vi "Connect-string.vi"(8 "error in (no error)":errorcluster caption="错误输入（无错误）", 10 "database-path":path, 11 "Database_access 输入":refnum<class "Database_access.lvclass">) -> (0 "error out":errorcluster caption="错误输出", 2 "connection reference":T1, 3 "Database_access 输出":refnum<class "Database_access.lvclass">)   [LabVIEW 2025, in "Database_access.lvclass"]
uses:
  Database_access.lvclass
  <vilib>/addons/database/Connection.llb/Conn ObjectReference.ctl
  Database_access.lvclass/Database_access.ctl
  <vilib>/addons/database/Connection.llb/DB Tools Open Connec (String).vi
  <vilib>/regexp/Match Regular Expression.xnode
  <vilib>/addons/database/NI_Database_API.lvlib
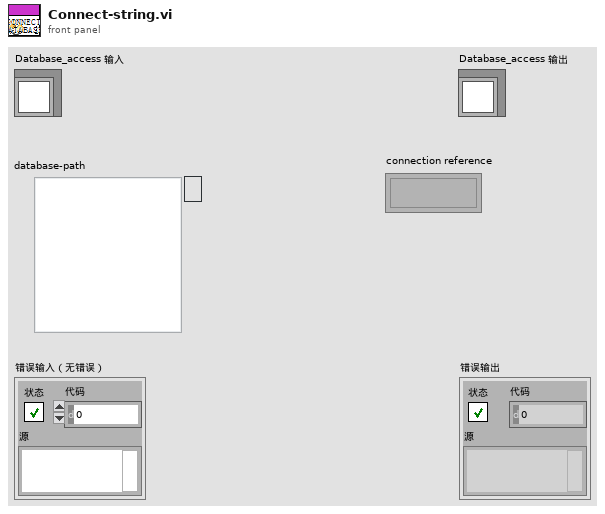
[diagram p1: front panel]
types:
  T1 = typedef "NI_Database_API.lvlib/Conn ObjectReference.ctl" = refnum<k1>
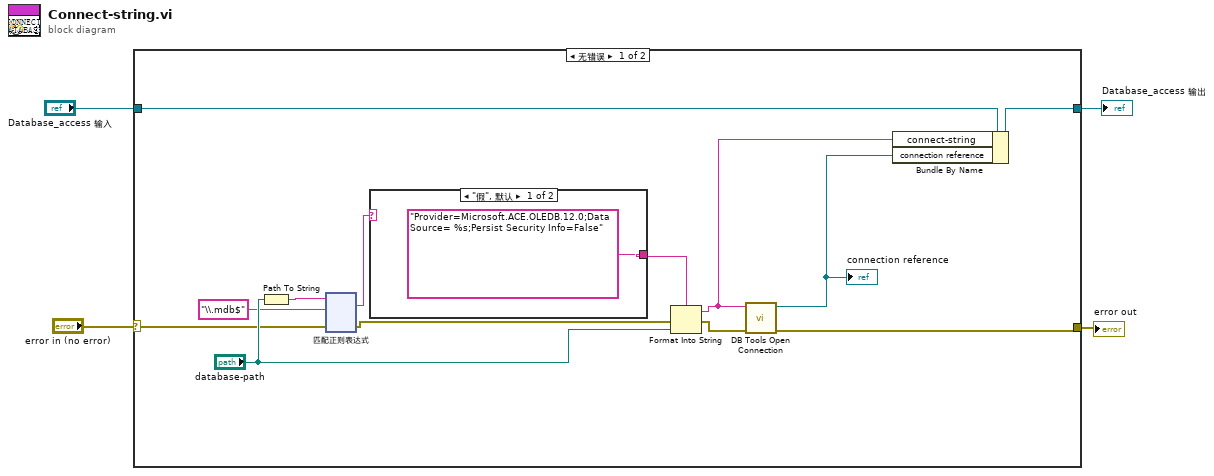
[diagram p0: block diagram]
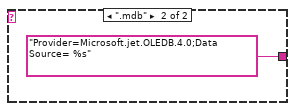
[diagram p2: hidden frame]
diagram:
  n1 = case shown="无错误" "error in (no error)" {
    selector: "error in (no error)" -> [w10 w138]
    tunnel: [w5 w138] -> w3
    tunnel: [w16 w137] -> w1
    tunnel: "Database_access 输入" -> [w17 w137]
    frame No Error {
      n2 = Path To String(path="database-path") -> (string=w12:string)
      n3 = xnode "匹配正则表达式"("输入字符串"=w12, "正则表达式"="\\.mdb$", "错误输入"=w10) -> ("所有匹配"=w9:string, "错误输出"=w8:errorcluster)  [unwired: 3 in, 3 out]
      n4 = case shown="\"假\", 默认" w9 {
        tunnel: ["Provider=Microsoft.ACE.OLEDB.12.0;Data Source= %s;Persist Security Info=False" "Provider=Microsoft.jet.OLEDB.4.0;Data Source= %s"] -> w7
        frame "假", Default {
        }
        frame ".mdb" {
        }
      }
      n5 = Format Into String(format string=w7, error in=w8, "database-path") -> (resulting string=w15:string, error out=w6:errorcluster)  [unwired: 1 in]
      n6 = call-poly <vilib>:"DB Tools Open Connection.vi"("error in (no error)"=w6, "connection information"=w15) -> ("error out"=w5:errorcluster, "connection reference"=w14:T1)  [unwired: 6 in]
      "connection reference" <- w14
      n7 = Bundle By Name(cluster=w17, "connect-string"=w15, "connection reference"=w14) -> (w16:refnum<class "Database_access.lvclass">)
    }
    frame Error {
    }
  }
  "error out" <- w3
  "Database_access 输出" <- w1
